vi "G_Variables.vi"() -> ()   [LabVIEW 2021, in "Simulator-Channel.lvlib"]
uses:
  Device Channels/Simulator/Channels/DIO-Channel/Simulator-Channel.lvlib
  <vilib>/ActorFramework/Message Enqueuer/Message Enqueuer.lvclass
panel:
  in  "AIO Actor":refnum<class "Message Enqueuer.lvclass">
  in  "DIO Actor":refnum<class "Message Enqueuer.lvclass">
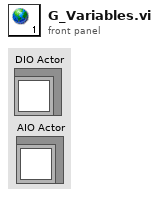
[diagram p1: front panel]
diagram:
